vi "[ce] LM Fit - get new coefficients.vi"(6 "lamda":dbl format="%.2e", 8 "error in":errorcluster, 9 "Beta":dbl[](array[numeric]) format="%.2f", 10 "Alpha":dbl[][](array[numeric]) format="%.2f", 11 "Coefficients":dbl[](array[numeric]) format="%.2f") -> (0 "error out":errorcluster, 2 "New Coefficients":dbl[](array[numeric]) format="%.2f", 3 "err flag":bool)   [LabVIEW 2021]
doc: "For computing new coefficients, this VI uses the 'get new coefficients.vi' VI located in 'labview\\vi.lib\\analysis\\6fits.llb'\n\n::: CalcExpress Toolkit :::\nCopyright (c) 2000-2026 Konstantin Shifershteyn. All rights reserved."
uses:
  <vilib>/Analysis/NI_AALPro.lvlib
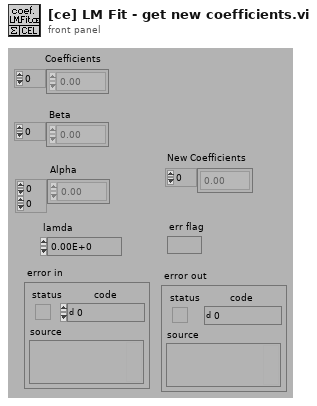
[diagram p1: front panel]
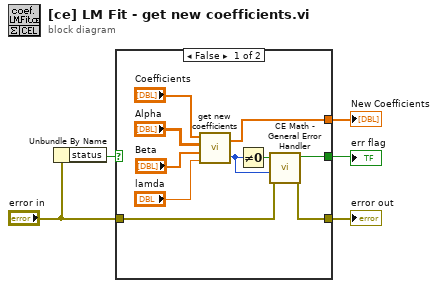
[diagram p0: block diagram]
diagram:
  n1 = Unbundle By Name("error in") -> ("status"=w3:bool)
  n2 = case shown="False" w3 {
    selector: w3 -> [_ w16]
    tunnel: [w6 _] -> w1
    tunnel: [w11 w17] -> w5
    tunnel: "error in" -> [w12 w17]
    tunnel: [w10 w16] -> w2
    frame False {
      n3 = call <vilib>:"get new coefficients.vi"("lamda"="lamda", "Beta"="Beta", "Alpha"="Alpha", "Coefficients"="Coefficients") -> ("error"=w8:i32, "New Coefficients"=w6:dbl[])
      n4 = Not Equal To 0?(x=w8) -> (x != 0?=w9:bool)
      n5 = call "CE Math - General Error Handler.vi"("error before"=w12, "error code"=w8, "error? (T)"=w9) -> ("error out"=w11:errorcluster, "error status"=w10:bool)  [unwired: 5 in]
    }
    frame True {
    }
  }
  "New Coefficients" <- w1
  "error out" <- w5
  "err flag" <- w2
